vi "process.vi"(8 "error in (no error)":errorcluster, 11 "ConnectionHandler in":refnum<class "ConnectionHandler.lvclass">) -> (0 "error out":errorcluster, 3 "ConnectionHandler":refnum<class "ConnectionHandler.lvclass">)   [LabVIEW 2013, in "MQTT Server.lvlib" / "ConnectionHandler.lvclass"]
uses:
  ConnectionHandler.lvclass
  <vilib>/LabVIEW Open Source Project/MQTT Connection/MQTT_Base/Session/Session.lvclass
  ConnectionHandler.lvclass/ConnectionHandler.ctl
  Session.Server/Session.Server.lvclass
  Client Event -- cluster.ctl
  Client Action -- enum.ctl
  <vilib>/LabVIEW Open Source Project/MQTT Connection/MQTT_Base/Session/Session.lvclass/Session.ctl
  <vilib>/Utility/error.llb/Clear Errors.vi
  <vilib>/LabVIEW Open Source Project/Connection/Connection/Connection.lvclass
panel:
  out "Stored Connections":i32
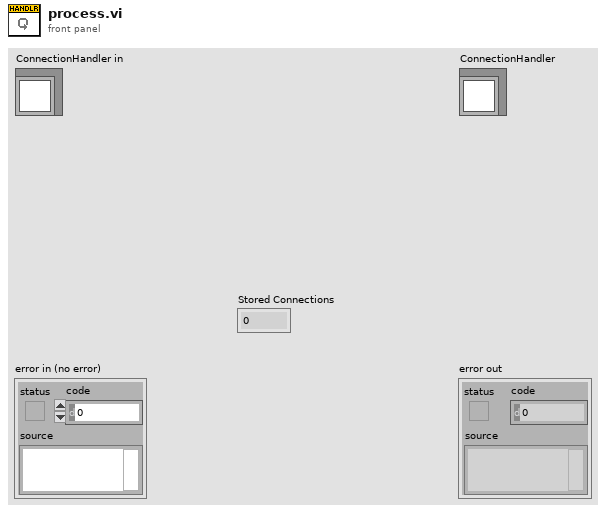
[diagram p1: front panel]
types:
  T1 = typedef "MQTT Server.lvlib/ConnectionHandler.lvclass/Client Event -- cluster.ctl" = cluster{"Action":T2, "Session ID":i32}
  T2 = typedef "MQTT Server.lvlib/ConnectionHandler.lvclass/Client Action -- enum.ctl" = enum16{"Connection", "Disconnection", "Session Stored", "Session Retrieved"}
  T3 = typedef "MQTT Server.lvlib/ConnectionHandler.lvclass/Public Events -- Cluster.ctl" = cluster{"NbConnections":refnum<user-event>, "ClientEvent":refnum<user-event>}
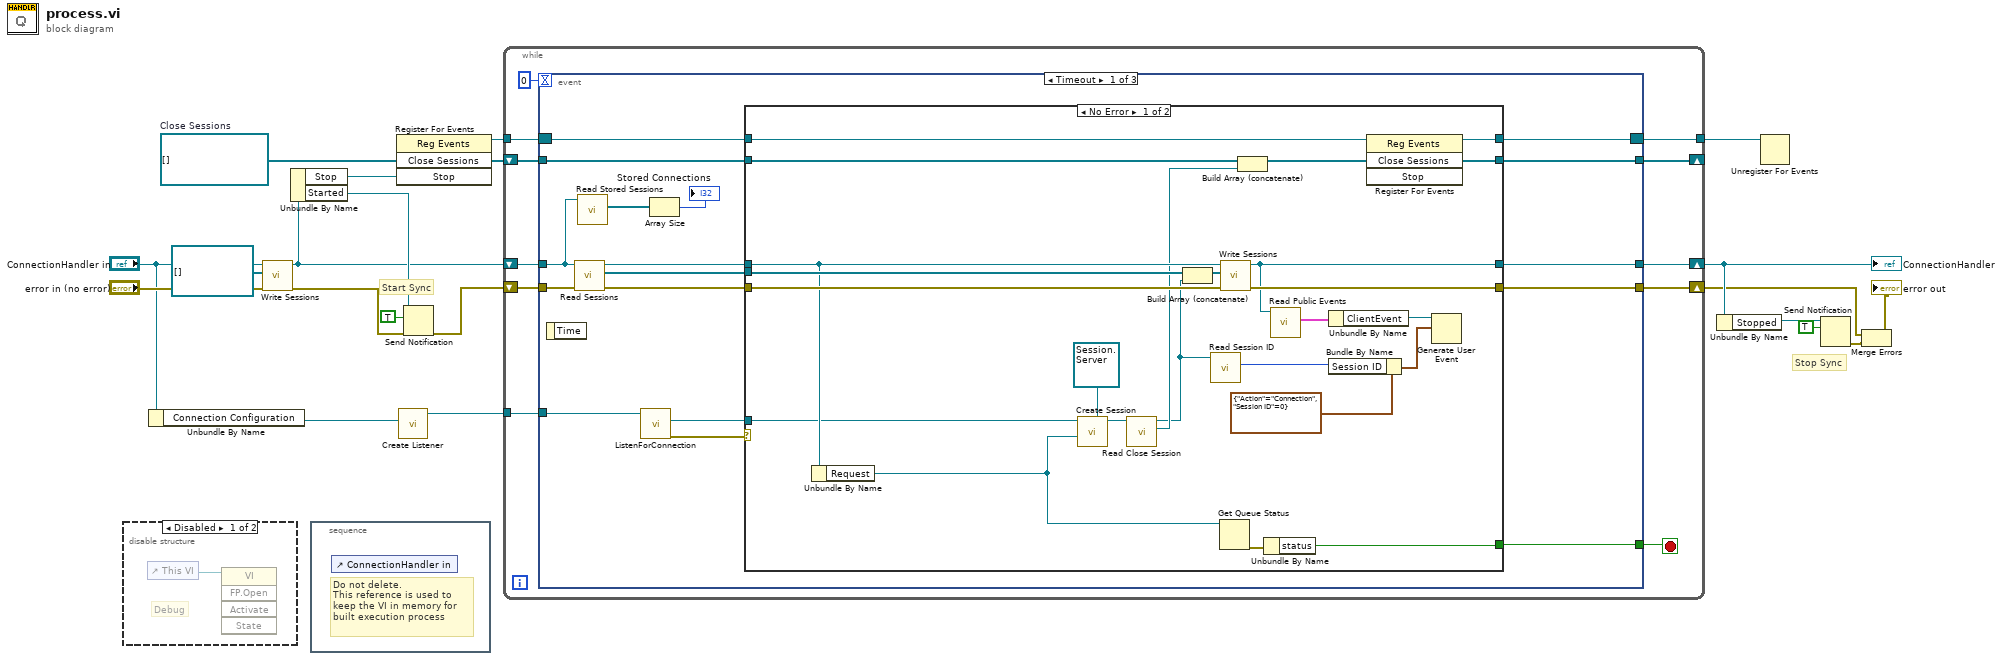
[diagram p0: block diagram]
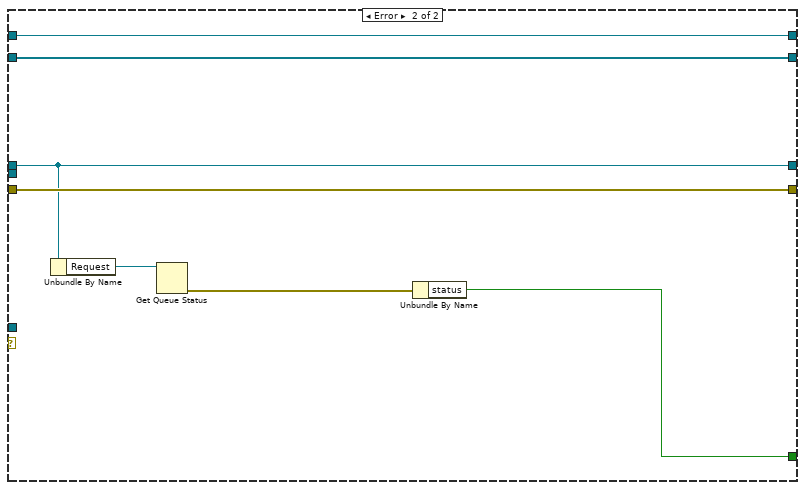
[diagram p3: hidden frame]
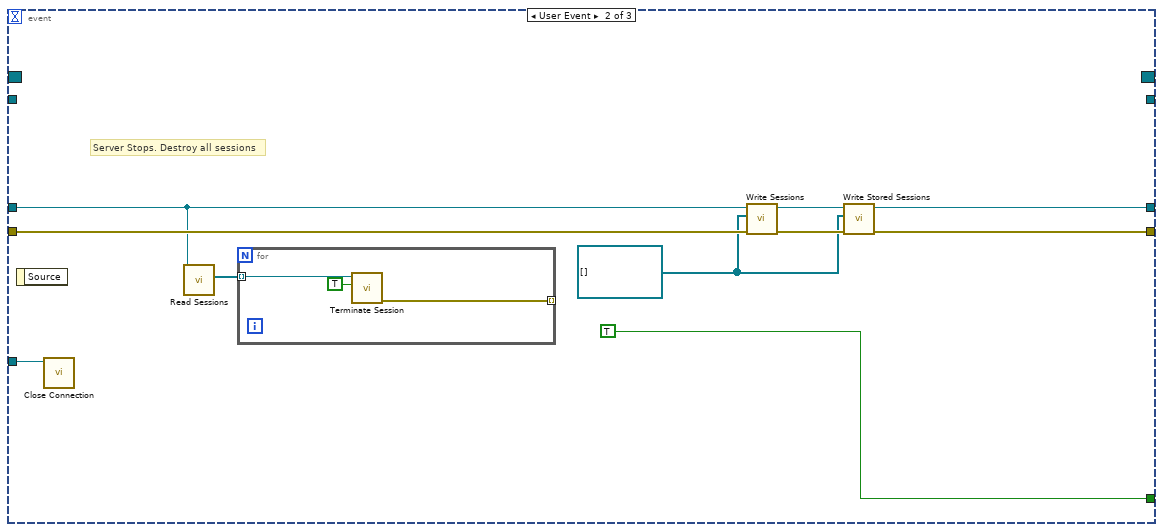
[diagram p4: hidden frame]
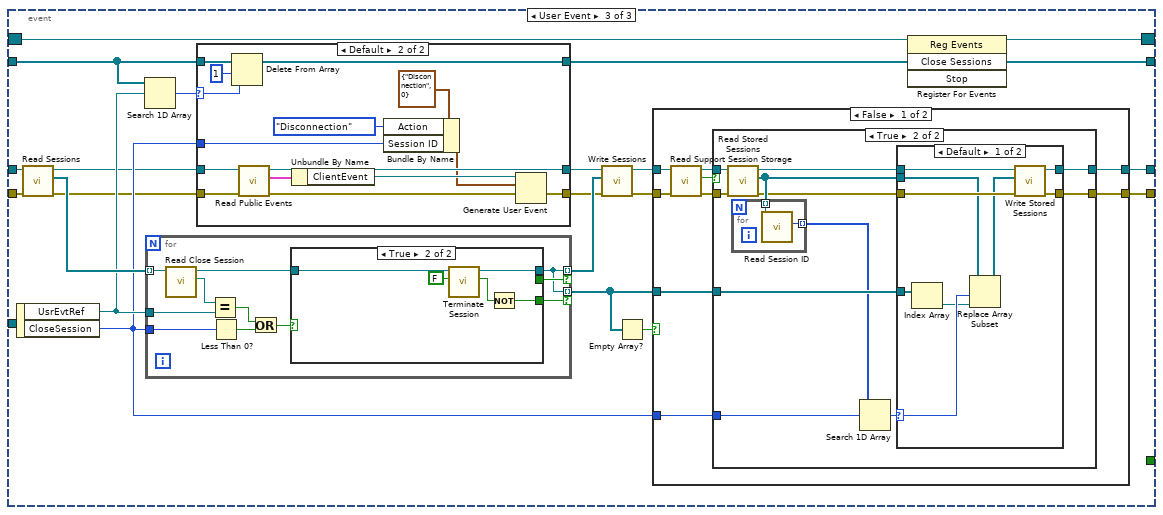
[diagram p5: hidden frame]
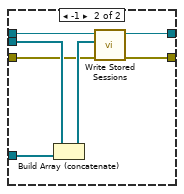
[diagram p8: hidden frame]
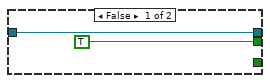
[diagram p10: hidden frame]
diagram:
  w4 = refnum<user-event>[] []  # Close Sessions
  # "Stop Sync"
  # "Start Sync"
  n1 = disable-structure shown="Disabled" {
    frame Disabled {
      # "Debug"
      n2 = control-ref of="This VI"() -> (w20:refnum<vi>)
      n3 = invoke class="VI" method="FP.Open"(reference=w20) -> ()  [unwired: 4 in, 5 out]
    }
    frame Enabled {
    }
  }
  n4 = Unbundle By Name("ConnectionHandler in") -> ("Connection Configuration"=w6:refnum<class "Connection.lvclass">)
  n5 = call "Write Sessions.vi"("Sessions"=refnum<class "Session.lvclass">[] [], "ConnectionHandler in"="ConnectionHandler in") -> ("ConnectionHandler"=w2:refnum<class "ConnectionHandler.lvclass">)  [unwired: 9 in]
  n6 = Unbundle By Name(w2) -> ("Stop"=w19:refnum<user-event>, "Started"=w14:refnum<notifier>)
  n7 = stacked-sequence {
    frame #0 {
      # "Do not delete.\nThis reference is used to keep the VI in memory for built execution process"
      n8 = control-ref of="ConnectionHandler in"() -> ()  [unwired: 1 out]
    }
  }
  n9 = register-events(w4, w19) -> (reference out=w17:refnum<event-registration>)  [unwired: 2 in, 1 out]
  n10 = call <vilib>:"Create Listener.vi"("Connection Configuration"=w6) -> ("Listener"=w5:refnum<class "Connection.lvclass">)  [unwired: 9 in, 1 out]
  n11 = Send Notification(notification=TRUE, notifier=w14, error in (no error)="error in (no error)") -> (error out=w15:errorcluster)  [unwired: 1 out]
  n12 = while {
    shift-right: [w28] -> w13
    shift-left: w2 -> [w27]
    shift-right: [w30] -> w8
    shift-left: w15 -> [w29]
    tunnel: w17 -> [w26]
    tunnel: [w25] -> w18
    tunnel: w5 -> [w23]
    shift-right: [w22] -> _
    shift-left: w4 -> [w21]
    stop <- w24 stop-if-true
    n13 = event shown="[0] Timeout" {
      selector: w26 -> [w35 _ w97]
      dyn-events: [w34 _ w98] -> w25
      timeout: 0 -> [_ _ _]
      tunnel: [w45 w84 w100] -> w30
      tunnel: w29 -> [w47 w84 w88]
      tunnel: [w46 w79 w104] -> w28
      tunnel: w27 -> [w41 w81 w93]
      tunnel: [w44 TRUE _] -> w24
      tunnel: w23 -> [w37 w77 _]
      tunnel: [w33 _ w94] -> w22
      tunnel: w21 -> [w32 _ w96]
      event Timeout {
        n14 = event-data() -> ()  [unwired: 1 in, 1 out]
        n15 = call "Read Sessions.vi"("ConnectionHandler in"=w41) -> ("Sessions"=w42:refnum<class "Session.lvclass">[], "ConnectionHandler"=w43:refnum<class "ConnectionHandler.lvclass">)  [unwired: 9 in]
        n16 = call "Read Stored Sessions.vi"("ConnectionHandler in"=w41) -> ("Stored Sessions"=w40:refnum<class "Session.lvclass">[])  [unwired: 9 in, 1 out]
        n17 = call <vilib>:"ListenForConnection.vi"("Listener"=w37) -> ("error out"=w38:errorcluster, "Connection"=w39:refnum<class "Connection.lvclass">)  [unwired: 7 in, 2 out]
        n18 = Array Size(array=w40) -> (size(s)=→"Stored Connections":i32)
        n19 = case shown="No Error" w38 {
          tunnel: w43 -> [w65 w75]
          tunnel: w47 -> [w69 w76]
          tunnel: [w54 w75] -> w46
          tunnel: [w69 w76] -> w45
          tunnel: [w67 w72] -> w44
          tunnel: w42 -> [w66 _]
          tunnel: w39 -> [w63 _]
          tunnel: w35 -> [w61 w71]
          tunnel: [w60 w71] -> w34
          tunnel: [w55 w70] -> w33
          tunnel: w32 -> [w56 w70]
          frame No Error {
            n20 = Unbundle By Name(w65) -> ("Request"=w62:refnum<queue>)
            n21 = call <vilib>:"Create Session.vi"("Session in"=refnum<class "Session.Server.lvclass"> refnum ("MQTT Server.lvlib:Session.Server.lvclass"), "Request"=w62, "Connection"=w63) -> ("Session"=w58:refnum<class "Session.Server.lvclass">)  [unwired: 7 in, 1 out]
            n22 = call <vilib>:"Read Close Session.vi"("Session in"=w58) -> ("Close Session"=w57:refnum<user-event>, "Session out"=w51:refnum<class "Session.Server.lvclass">)  [unwired: 8 in, 1 out]
            n23 = Build Array (concatenate)(w66, w51) -> (w59:refnum<class "Session.lvclass">[])
            n24 = call <vilib>:"Read Session ID.vi"("Session in"=w51) -> ("Session ID"=w49:i32)  [unwired: 8 in, 2 out]
            n25 = Get Queue Status(queue=w62) -> (error out=w68:errorcluster)  [unwired: 2 in, 7 out]
            n26 = call "Write Sessions.vi"("Sessions"=w59, "ConnectionHandler in"=w65) -> ("ConnectionHandler"=w54:refnum<class "ConnectionHandler.lvclass">)  [unwired: 9 in]
            n27 = Build Array (concatenate)(w56, w57) -> (w55:refnum<user-event>[])
            n28 = Unbundle By Name(w68) -> ("status"=w67:bool)
            n29 = call "Read Public Events.vi"("TCPConnectionHandler in"=w54) -> ("Connection Handler Public Events"=w53:T3)  [unwired: 8 in, 2 out]
            n30 = Unbundle By Name(w53) -> ("ClientEvent"=w52:refnum<user-event>)
            n31 = Bundle By Name(cluster=T1 {"Action"=enum."Connection", "Session ID"=0} ("Client Event"), "Session ID"=w49) -> (w48:T1)
            n32 = register-events(reference=w61, w55) -> (reference out=w60:refnum<event-registration>)  [unwired: 2 in, 1 out]
            n33 = Generate User Event(user event=w52, event data cluster=w48) -> ()  [unwired: 2 in, 2 out]
          }
          frame Error {
            n34 = Unbundle By Name(w75) -> ("Request"=w74:refnum<queue>)
            n35 = Get Queue Status(queue=w74) -> (error out=w73:errorcluster)  [unwired: 2 in, 7 out]
            n36 = Unbundle By Name(w73) -> ("status"=w72:bool)
          }
        }
      }
      event User Event {
        w78 = refnum<class "Session.lvclass">[] [] ("Sessions")
        # "Server Stops. Destroy all sessions"
        n37 = event-data() -> ()  [unwired: 1 in, 1 out]
        n38 = call <vilib>:"Close Connection.vi"("Connection in"=w77) -> ()  [unwired: 9 in, 2 out]
        n39 = call "Read Sessions.vi"("ConnectionHandler in"=w81) -> ("Sessions"=w82:refnum<class "Session.lvclass">[])  [unwired: 9 in, 1 out]
        n40 = for {
          tunnel: w82 -> [w87] mode=indexing
          tunnel: [w86] -> _ mode=indexing
          n41 = call <vilib>:"Terminate Session.vi"("Destroy (T)"=TRUE, "Session in"=w87) -> ("error out"=w86:errorcluster)  [unwired: 7 in, 2 out]
        }
        n42 = call "Write Sessions.vi"("Sessions"=w78, "ConnectionHandler in"=w81) -> ("ConnectionHandler"=w80:refnum<class "ConnectionHandler.lvclass">)  [unwired: 9 in]
        n43 = call "Write Stored Sessions.vi"("Stored Sessions"=w78, "ConnectionHandler in"=w80) -> ("ConnectionHandler"=w79:refnum<class "ConnectionHandler.lvclass">)  [unwired: 9 in]
      }
      event User Event {
        n44 = event-data() -> ("UsrEvtRef"=w99:refnum<user-event>, "CloseSession"=w92:i32)  [unwired: 1 in]
        n45 = call "Read Sessions.vi"("ConnectionHandler in"=w93) -> ("Sessions"=w106:refnum<class "Session.lvclass">[], "ConnectionHandler"=w91:refnum<class "ConnectionHandler.lvclass">)  [unwired: 9 in]
        n46 = Search 1D Array(1D array=w96, element=w99) -> (index of element=w95:i32)  [unwired: 1 in]
        n47 = for {
          tunnel: w106 -> [w164] mode=indexing
          tunnel: [w170] -> w105 mode=indexing if=w174
          tunnel: w92 -> [w172]
          tunnel: [w170] -> w102 mode=indexing if=w169
          tunnel: w99 -> [w167]
          n48 = call <vilib>:"Read Close Session.vi"("Session in"=w164) -> ("Close Session"=w165:refnum<user-event>, "Session out"=w168:refnum<class "Session.lvclass">)  [unwired: 8 in, 1 out]
          n49 = Equal?(x=w165, y=w167) -> (x = y?=w166:bool)
          n50 = Less Than 0?(x=w172) -> (x < 0?=w173:bool)
          n51 = Or(x=w166, y=w173) -> (x .or. y?=w171:bool)
          n52 = case shown="True" w171 {
            tunnel: w168 -> [w176 w181]
            tunnel: [w176 w180] -> w170
            tunnel: [TRUE _] -> w174
            tunnel: [_ w177] -> w169
            frame False {
            }
            frame True {
              n53 = call <vilib>:"Terminate Session.vi"("Destroy (T)"=FALSE, "Session in"=w181) -> ("Destroyed"=w178:bool, "Session out"=w180:refnum<class "Session.lvclass">)  [unwired: 7 in, 1 out]
              n54 = Not(x=w178) -> (.not. x?=w177:bool)
            }
          }
        }
        n55 = case shown="Default" w95 {
          selector: w95 -> [_ w121]
          tunnel: w96 -> [w109 w124]
          tunnel: [w109 w122] -> w94
          tunnel: w92 -> [_ w114]
          tunnel: w91 -> [w108 w117]
          tunnel: [w108 w115] -> w90
          tunnel: [w107 w110] -> w89
          tunnel: w88 -> [w107 w113]
          frame -1 {
          }
          frame Default {
            n56 = Delete From Array(array=w124, length=1, index=w121) -> (array with subset deleted=w122:refnum<user-event>[])  [unwired: 1 out]
            n57 = call "Read Public Events.vi"("error in (no error)"=w113, "TCPConnectionHandler in"=w117) -> ("error out"=w111:errorcluster, "Connection Handler Public Events"=w118:T3, "TCPConnectionHandler out"=w115:refnum<class "ConnectionHandler.lvclass">)  [unwired: 7 in]
            n58 = Unbundle By Name(w118) -> ("ClientEvent"=w119:refnum<user-event>)
            n59 = Bundle By Name(cluster=T1 {"Action"=enum."Disconnection", "Session ID"=0} ("Client Event"), "Action"=Client_Action_--_enum."Disconnection", "Session ID"=w114) -> (w112:T1)
            n60 = Generate User Event(user event=w119, event data cluster=w112, error in=w111) -> (error out=w110:errorcluster)  [unwired: 1 in, 1 out]
          }
        }
        n61 = call "Write Sessions.vi"("Sessions"=w105, "ConnectionHandler in"=w90) -> ("ConnectionHandler"=w103:refnum<class "ConnectionHandler.lvclass">)  [unwired: 9 in]
        n62 = Empty Array?(array=w102) -> (empty?=w101:bool)
        n63 = case shown="False" w101 {
          tunnel: [w133 w163] -> w104
          tunnel: w103 -> [w129 w163]
          tunnel: w102 -> [w132 _]
          tunnel: [w130 w162] -> w100
          tunnel: w89 -> [w127 w162]
          tunnel: w92 -> [w131 _]
          frame False {
            n64 = call "Read Support Session Storage.vi"("error in (no error)"=w127, "ConnectionHandler in"=w129) -> ("error out"=w126:errorcluster, "Support Session Storage"=w125:bool, "ConnectionHandler out"=w128:refnum<class "ConnectionHandler.lvclass">)  [unwired: 7 in]
            n65 = case shown="True" w125 {
              tunnel: [w135 w145] -> w133
              tunnel: w132 -> [_ w143]
              tunnel: w131 -> [_ w140]
              tunnel: [w134 w138] -> w130
              tunnel: w128 -> [w135 w137]
              tunnel: w126 -> [w134 w136]
              frame False {
              }
              frame True {
                n66 = call "Read Stored Sessions.vi"("ConnectionHandler in"=w137) -> ("Stored Sessions"=w142:refnum<class "Session.lvclass">[], "ConnectionHandler"=w144:refnum<class "ConnectionHandler.lvclass">)  [unwired: 9 in]
                n67 = for {
                  tunnel: w142 -> [w161] mode=indexing
                  tunnel: [w160] -> w141 mode=indexing
                  n68 = call <vilib>:"Read Session ID.vi"("Session in"=w161) -> ("Session ID"=w160:i32)  [unwired: 8 in, 2 out]
                }
                n69 = Search 1D Array(1D array=w141, element=w140) -> (index of element=w139:i32)  [unwired: 1 in]
                n70 = case shown="Default" w139 {
                  selector: w139 -> [w149 _]
                  tunnel: [w153 w159] -> w145
                  tunnel: w144 -> [w151 w158]
                  tunnel: w143 -> [w148 w156]
                  tunnel: w142 -> [w150 w155]
                  tunnel: w136 -> [w152 w154]
                  tunnel: [w152 w154] -> w138
                  frame Default {
                    n71 = Index Array(array=w148) -> (element=w147:refnum<class "Session.lvclass">)  [unwired: 1 in]
                    n72 = Replace Array Subset(array=w150, new element=w147, index=w149) -> (w146:refnum<class "Session.lvclass">[])
                    n73 = call "Write Stored Sessions.vi"("Stored Sessions"=w146, "ConnectionHandler in"=w151) -> ("ConnectionHandler"=w153:refnum<class "ConnectionHandler.lvclass">)  [unwired: 9 in]
                  }
                  frame -1 {
                    n74 = Build Array (concatenate)(w155, w156) -> (w157:refnum<class "Session.lvclass">[])
                    n75 = call "Write Stored Sessions.vi"("Stored Sessions"=w157, "ConnectionHandler in"=w158) -> ("ConnectionHandler"=w159:refnum<class "ConnectionHandler.lvclass">)  [unwired: 9 in]
                  }
                }
              }
            }
          }
          frame True {
          }
        }
        n76 = register-events(reference=w97, w94) -> (reference out=w98:refnum<event-registration>)  [unwired: 2 in, 1 out]
      }
    }
  }
  "ConnectionHandler" <- w13
  n77 = Unbundle By Name(w13) -> ("Stopped"=w12:refnum<notifier>)
  n78 = Unregister For Events(event registration refnum=w18) -> ()  [unwired: 1 in, 1 out]
  n79 = Send Notification(notification=TRUE, notifier=w12) -> (error out=w9:errorcluster)  [unwired: 1 in, 1 out]
  n80 = Merge Errors(w8, w9) -> (→"error out":errorcluster)
